vi "Set Reentrant.vi"() -> ()   [LabVIEW 2020]
doc: "Build helper: makes the VI at path reentrant (Exec.IsReentrant TRUE) and saves it; reports the reentrancy type before and after."
panel:
  out "summary":string
  in  "path":path
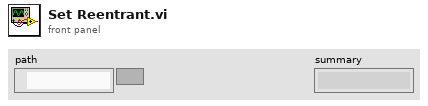
[diagram p1: front panel]
types:
  T1 = enum16{"Share clones between instances", "Preallocate clone for each instance"}
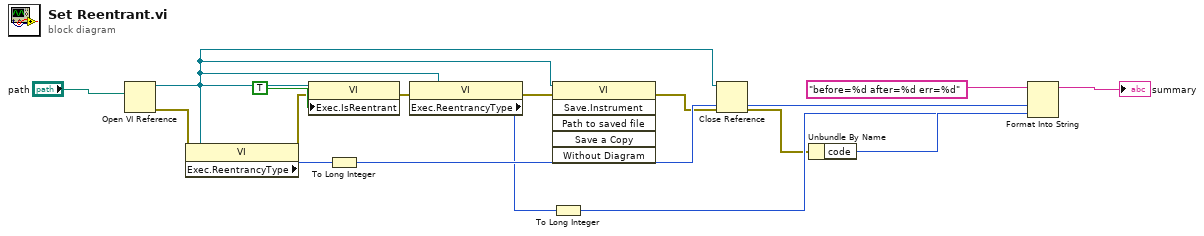
[diagram p0: block diagram]
diagram:
  n1 = Open VI Reference(vi path="path") -> (vi reference=w2:refnum<vi>, error out=w3:errorcluster)  [unwired: 5 in]
  n2 = property class="VI"(reference=w2, error in=w3) -> (error out=w5:errorcluster, "Exec.ReentrancyType"=w4:T1)  [unwired: 1 out]
  n3 = property class="VI"(reference=w2, error in=w5, "Exec.IsReentrant"=TRUE) -> (error out=w7:errorcluster)  [unwired: 1 out]
  n4 = To Long Integer(number=w4) -> (32bit integer=w12:i32)
  n5 = property class="VI"(reference=w2, error in=w7) -> (error out=w9:errorcluster, "Exec.ReentrancyType"=w8:T1)  [unwired: 1 out]
  n6 = invoke class="VI" method="Save.Instrument"(reference=w2, error in=w9) -> (error out=w10:errorcluster)  [unwired: 4 in, 5 out]
  n7 = To Long Integer(number=w8) -> (32bit integer=w13:i32)
  n8 = Close Reference(reference=w2, error in (no error)=w10) -> (error out=w11:errorcluster)
  n9 = Unbundle By Name(w11) -> ("code"=w14:i32)
  n10 = Format Into String(format string="before=%d after=%d err=%d", w12, w13, w14) -> (resulting string=→"summary":string)  [unwired: 2 in, 1 out]
